vi "Channels.vi"() -> (2 "Names":string[](array[string]), 3 "Channels to Create":T1[](array[typedef]) {"Custom Config Data" format="%x"})   [LabVIEW 2021, in "CAN_Reader_NIXNET_Common.lvlib"]
uses:
  CAN_Reader_NIXNET_Common.lvlib
  <vilib>/CIF Foundation/CIF Core/Channels/ChannelRegistrar/typedef/Channel Definition.ctl
  <vilib>/CIF Foundation/CIF Channels Core/ChannelCommon/typedef/Direction.ctl
  <vilib>/CIF Foundation/CIF Core/Channels/ChannelRegistrar/typedef/Registered Channel Types.ctl
  <vilib>/CIF Foundation/CIF Channels Core/ChannelCommon/typedef/New FIFO Config.ctl
  <vilib>/CIF Foundation/CIF Channels Core/ChannelCommon/typedef/FIFO Flags.ctl
  <vilib>/CIF Foundation/CIF Core/Channels/ChannelRegistrar/ChannelRegistrar.lvlib
  <vilib>/CIF Foundation/CIF Channels Core/ChannelCommon/ChannelCommon.lvlib
  <vilib>/CIF Foundation/CIF LabVIEW Scripting/Update Enum/Update Enum.lvlib
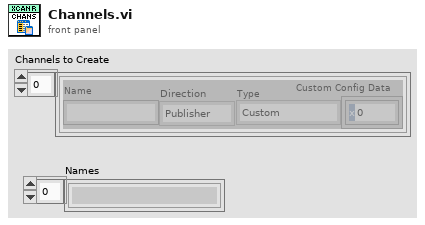
[diagram p1: front panel]
types:
  T1 = typedef "ChannelRegistrar.lvlib/Channel Definition.ctl" = cluster{"Name":string, "Direction":T2, "Type":T3, "Custom Config Data":u8[]}
  T2 = typedef "ChannelCommon.lvlib/Direction.ctl" = enum8{"Publisher", "Subscriber"}
  T3 = typedef "ChannelRegistrar.lvlib/Registered Channel Types.ctl" = enum8{"Custom", "Double_Tag", "I64_Tag", "U64_Tag", "U8_FIFO", "CAN_FIFO", "L2Enet_FIFO", "DAQ_FIFO", "Universal_FIFO", "String_Tag"}
  T4 = typedef "ChannelCommon.lvlib/New FIFO Config.ctl" = cluster{"Max Bytes/Msg":u64, "Max Msg/FIFO":u64, "FIFO Flags":T5}
  T5 = typedef "ChannelCommon.lvlib/FIFO Flags.ctl" = cluster{"Backpressure":bool}
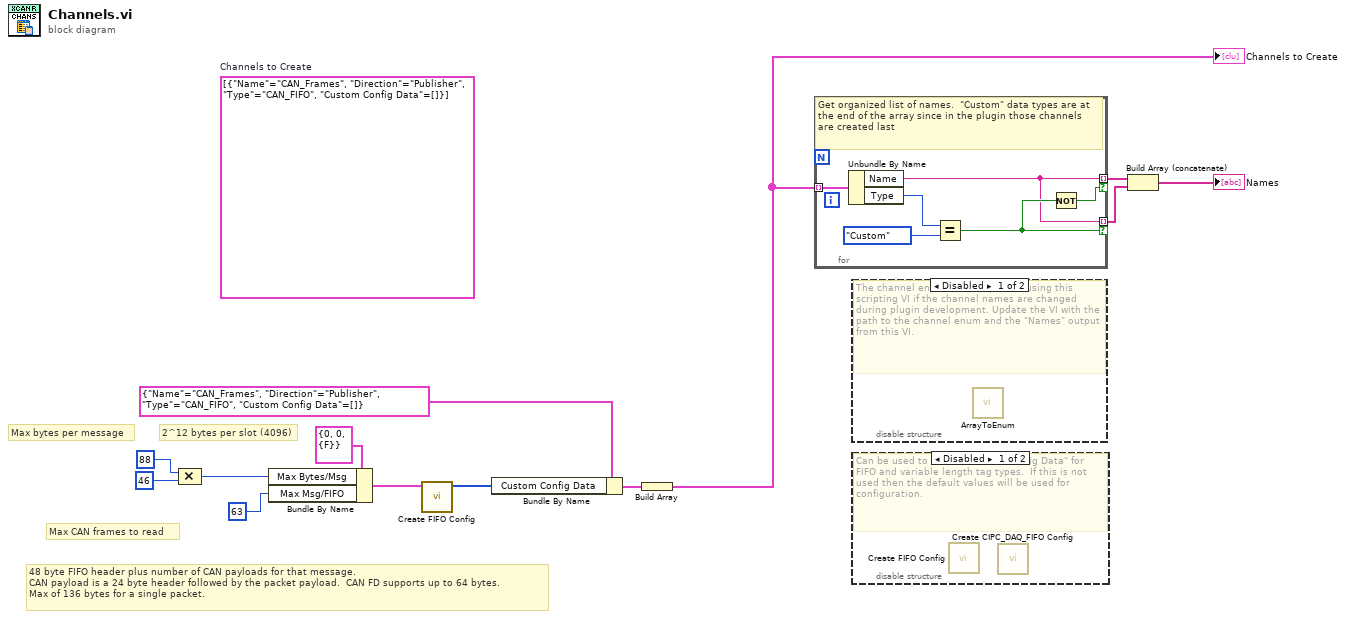
[diagram p0: block diagram]
diagram:
  (unwired) T1[] [{"Name"="CAN_Frames", "Direction"=enum."Publisher", "Type"=enum."CAN_FIFO", "Custom Config Data"=[]}]  # Channels to Create
  # "2^12 bytes per slot (4096)"
  # "48 byte FIFO header plus number of CAN payloads for that message.\nCAN payload is a 24 byte header followed by the packet payload.  CAN FD supports up to 64 bytes.\nMax of 136 bytes for a single packet."
  # "Max bytes per message"
  # "Max CAN frames to read"
  n1 = Compound Arithmetic op=MULTIPLY(u64 88 ("Max Msg/FIFO"), u64 46 ("value")) -> (w1:u64)
  n2 = Bundle By Name(cluster=T4 {"Max Bytes/Msg"=0, "Max Msg/FIFO"=0, "FIFO Flags"={"Backpressure"=FALSE}} ("New FIFO Config"), "Max Bytes/Msg"=w1, "Max Msg/FIFO"=u64 63) -> (w8:T4)
  n3 = call <vilib>:"Create FIFO Config.vi"("New FIFO Config"=w8) -> ("Flattened FIFO Config"=w9:u8[])  [unwired: 10 in]
  n4 = Bundle By Name(cluster=T1 {"Name"="CAN_Frames", "Direction"=enum."Publisher", "Type"=enum."CAN_FIFO", "Custom Config Data"=[]} ("Channel Definition"), "Custom Config Data"=w9) -> (w3:T1)
  n5 = Build Array(w3) -> (w2:T1[])
  "Channels to Create" <- w2
  n6 = for {
    tunnel: w2 -> [w19] mode=indexing
    tunnel: [w14] -> w13 mode=indexing if=w15
    tunnel: [w14] -> w12 mode=indexing if=w16
    # "Get organized list of names.  \"Custom\" data types are at the end of the array since in the plugin those channels are created last"
    n7 = Unbundle By Name(w19) -> ("Name"=w14:string, "Type"=w18:T3)
    n8 = Equal?(x=w18, y=Registered_Channel_Types."Custom") -> (x = y?=w16:bool)
    n9 = Not(x=w16) -> (.not. x?=w15:bool)
  }
  n10 = disable-structure shown="Disabled" {
    frame Disabled {
      # "The channel enum can be updated using this scripting VI if the channel names are changed during plugin development. Update the VI with the path to the channel enum and the \"Names\" output from this VI."
      n11 = call <vilib>:"ArrayToEnum.vi"() -> ()  [unwired: 11 in, 1 out]
    }
    frame Enabled {
    }
  }
  n12 = disable-structure shown="Disabled" {
    frame Disabled {
      # "Can be used to create \"Custom Config Data\" for FIFO and variable length tag types.  If this is not used then the default values will be used for configuration."
      n13 = call <vilib>:"Create FIFO Config.vi"() -> ()  [unwired: 11 in, 1 out]
      n14 = call <vilib>:"Create CIPC_DAQ_FIFO Config.vi"() -> ()  [unwired: 11 in, 1 out]
    }
    frame Enabled {
    }
  }
  n15 = Build Array (concatenate)(w13, w12) -> (→"Names":string[])
